vi "GetTestDataValuePrecision.vi"(4 "TestMode":enum16{"電子中軸測試", "中置電機測試"}(ring), 5 "Wiring":u16) -> (1 "Boolean":bool, 2 "Procisions":i32[](array[numeric]))   [LabVIEW 2024]
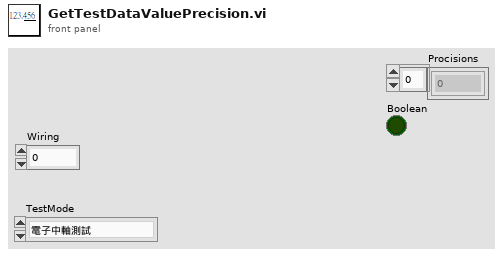
[diagram p1: front panel]
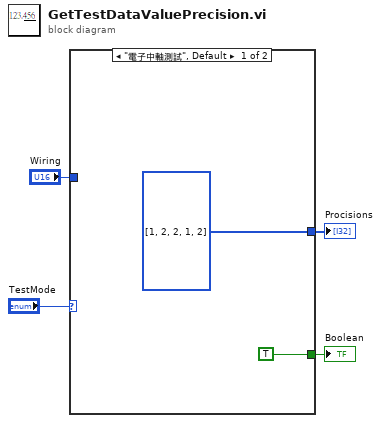
[diagram p0: block diagram]
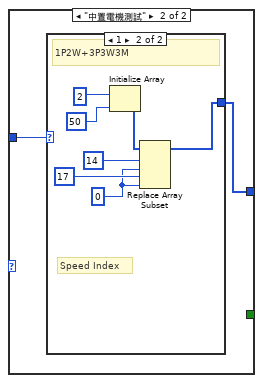
[diagram p2: hidden frame]
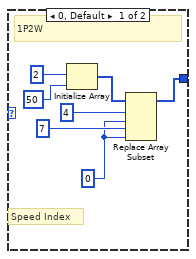
[diagram p3: hidden frame]
diagram:
  n1 = case shown="\"電子中軸測試\", Default" "TestMode" {
    tunnel: "Wiring" -> [_ w8]
    tunnel: [i32[] [1, 2, 2, 1, 2] w7] -> w2
    tunnel: [TRUE _] -> w1
    frame "電子中軸測試", Default {
    }
    frame "中置電機測試" {
      n2 = case shown="1" w8 {
        tunnel: [w11 w16] -> w7
        frame 0, Default {
          w9 = 0 ("new element/subarray")
          # "Speed Index"
          # "1P2W"
          n3 = Initialize Array(2, 50 ("dimension size")) -> (w13:i32[])
          n4 = Replace Array Subset(array=w13, new element #1=w9, index #1=4 ("index"), new element #2=w9, index #2=7 ("index")) -> (w11:i32[])
        }
        frame 1 {
          w17 = 0 ("new element/subarray")
          # "Speed Index"
          # "1P2W+3P3W3M"
          n5 = Initialize Array(2, 50 ("dimension size")) -> (w20:i32[])
          n6 = Replace Array Subset(array=w20, new element #1=w17, index #1=14 ("index"), new element #2=w17, index #2=17 ("index")) -> (w16:i32[])
        }
      }
    }
  }
  "Procisions" <- w2
  "Boolean" <- w1
